vi "Get ACS status.vi"(8 "error in (no error)":errorcluster, 11 "SPARC4_GEI in":refnum<class "S4GEI.lvclass">) -> (0 "error out":errorcluster, 3 "SPARC4_GEI out":refnum<class "S4GEI.lvclass">)   [LabVIEW 2018, in "S4GEI.lvclass"]
uses:
  S4GEI.lvclass
  S4GEI.lvclass/S4GEI.ctl
  Channel GUI/Channel.lvclass
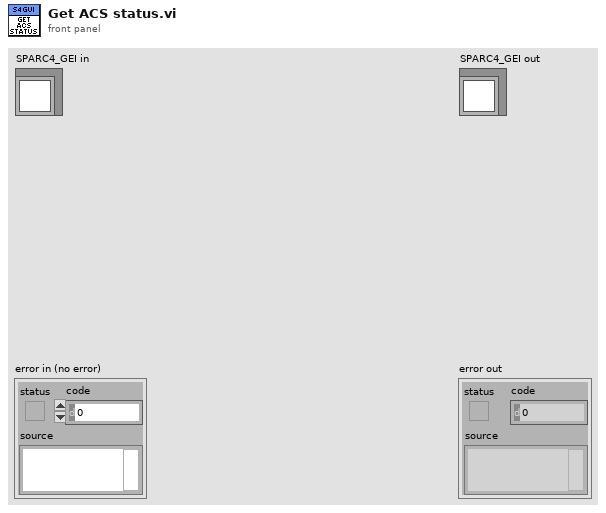
[diagram p1: front panel]
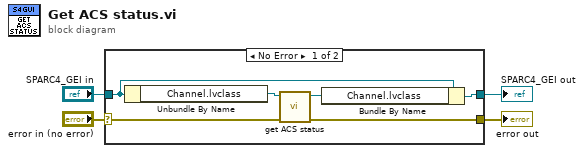
[diagram p0: block diagram]
diagram:
  n1 = case shown="No Error" "error in (no error)" {
    selector: "error in (no error)" -> [w10 w12]
    tunnel: [w9 w12] -> w3
    tunnel: [w5 w11] -> w1
    tunnel: "SPARC4_GEI in" -> [w6 w11]
    frame No Error {
      n2 = Unbundle By Name(w6) -> ("Channel.lvclass"=w8:refnum<class "Channel.lvclass">)
      n3 = call "get ACS status.vi"("error in (no error)"=w10, "Channel in"=w8) -> ("error out"=w9:errorcluster, "Channel out"=w7:refnum<class "Channel.lvclass">)  [unwired: 8 in]
      n4 = Bundle By Name(cluster=w6, "Channel.lvclass"=w7) -> (w5:refnum<class "S4GEI.lvclass">)
    }
    frame Error {
    }
  }
  "error out" <- w3
  "SPARC4_GEI out" <- w1
